vi "SUP_Camera_Queue_Latest.vi"(11 "packet":variant) -> (0 "telemetry error":errorcluster caption="sortie d'erreur", 3 "replaced_or_error":bool)   [LabVIEW 2012]
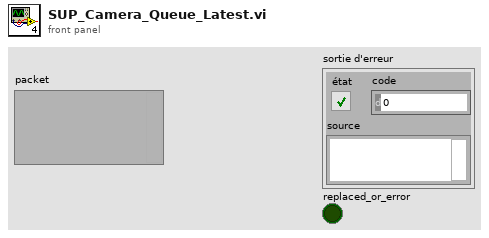
[diagram p1: front panel]
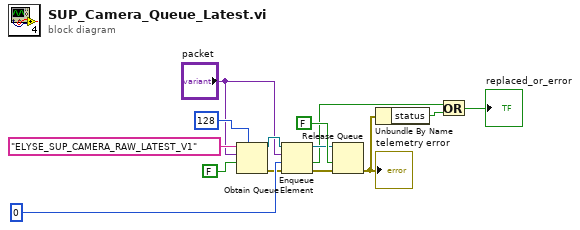
[diagram p0: block diagram]
diagram:
  n1 = Obtain Queue(max queue size (-1, unlimited)=128 ("taille max de la file d'attente (-1, non limitée)"), name (unnamed)="ELYSE_SUP_CAMERA_RAW_LATEST_V1" ("nom (aucun)"), element data type="packet", create if not found? (T)=FALSE ("créer si introuvable ? (V)")) -> (queue out=w7:refnum<queue>, error out=w4:errorcluster)  [unwired: 1 in, 1 out]
  n2 = Enqueue Element(queue=w7, element="packet", timeout in ms (-1)=0 ("timeout en ms (-1)"), error in (no error)=w4) -> (queue out=w3:refnum<queue>, timed out?=w1:bool, error out=w2:errorcluster)
  n3 = Release Queue(queue=w3, force destroy? (F)=FALSE ("forcer la destruction ? (F)"), error in (no error)=w2) -> (error out=w10:errorcluster)  [unwired: 2 out]
  "telemetry error" <- w10
  n4 = Unbundle By Name(w10) -> ("status"=w9:bool)
  n5 = Or(x=w1, y=w9) -> (x .or. y?=→"replaced_or_error":bool)
